vi "GetGrabberPositions.vi"(0 "reference":refnum<class "PackageNode.lvclass">, 5 "error in (no error)":errorcluster) -> (14 "reference out":refnum<class "PackageNode.lvclass">, 15 "GrabberPositions":T2[](array[typedef]) {"y" format="%.2f"; "x" format="%.2f"}, 16 "HotSpots":T1[](array[typedef]) {"HotSpot"."y" format="%.2f"; "HotSpot"."x" format="%.2f"}, 19 "error out":errorcluster)   [LabVIEW 2020, in "PackageNode.lvclass"]
doc: "public Rectangle2D getBounds(Graphics2D g2)"
uses:
  <resource>/Framework/Providers/Open_GDS/UML/PackageNode_class/PackageNode.lvclass
  C:/Program Files (x86)/National Instruments/LabVIEW 2020/resource/Framework/Providers/Open_GDS/UML/RectangularNode_class/RectangularNode.lvclass
  C:/Program Files (x86)/National Instruments/LabVIEW 2020/resource/Framework/Providers/Open_GDS/UML/AbstractNode_class/AbstractNode.lvclass
  <resource>/Framework/Providers/Open_GDS/UML/General/Point/Point Point2D.ctl
  <resource>/Framework/Providers/Open_GDS/UML/UMLEditor/UMLEditor_HotSpotData.ctl
  <resource>/Framework/Providers/Open_GDS/UML/AbstractNode_class/AbstractNode.lvclass
  <resource>/Framework/Providers/Open_GDS/UML/UMLEditor/UMLEditor_HotSpotType.ctl
  <resource>/Framework/Providers/Open_GDS/UML/RectangularNode_class/RectangularNode.lvclass
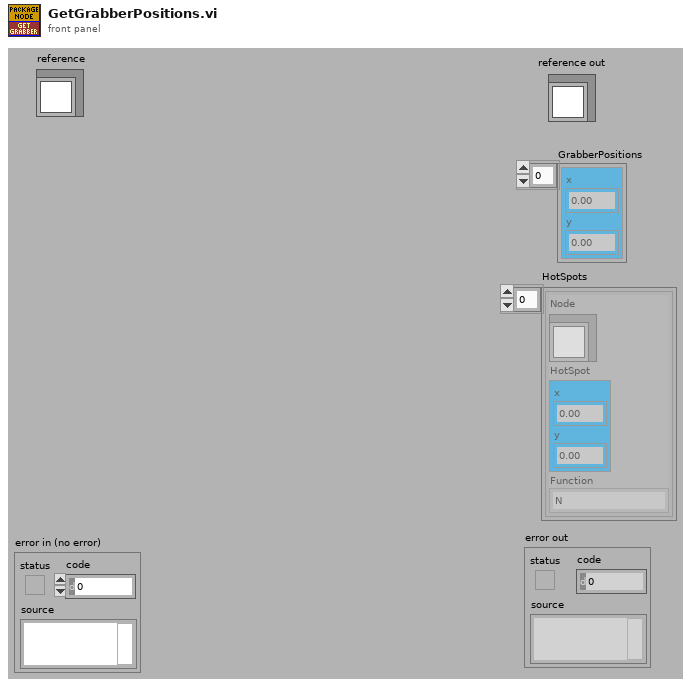
[diagram p1: front panel]
types:
  T1 = typedef "UMLEditor_HotSpotData.ctl" = cluster{"Node":refnum<class "AbstractNode.lvclass">, "HotSpot":T2, "Function":T3}
  T2 = typedef "Point Point2D.ctl" = cluster{"x":dbl, "y":dbl}
  T3 = typedef "UMLEditor_HotSpotType.ctl" = enum16{"N", "NE", "E", "SE", "S", "SW", "W", "NW", "Expand", "Collaps"}
  T4 = typedef "PackageNode.lvclass/ObjectAttributes.ctl" = cluster{"name":string, "contents":refnum<class "MultiLineString.lvclass">, "DEFAULT_TOP_WIDTH":i32, "DEFAULT_TOP_HEIGHT":i32, "DEFAULT_WIDTH":i32, "DEFAULT_HEIGHT":i32, "NAME_GAP":i32, "XGAP":i32, "YGAP":i32, "Collapsed":bool, "Note color":u32, "Justification":u16}
  T5 = typedef "RectangularNode.lvclass/ObjectAttributes.ctl" = cluster{"bounds":T6}
  T6 = typedef "Rectangle Rectangle2D.ctl" = cluster{"x":dbl, "y":dbl, "width":dbl, "height":dbl}
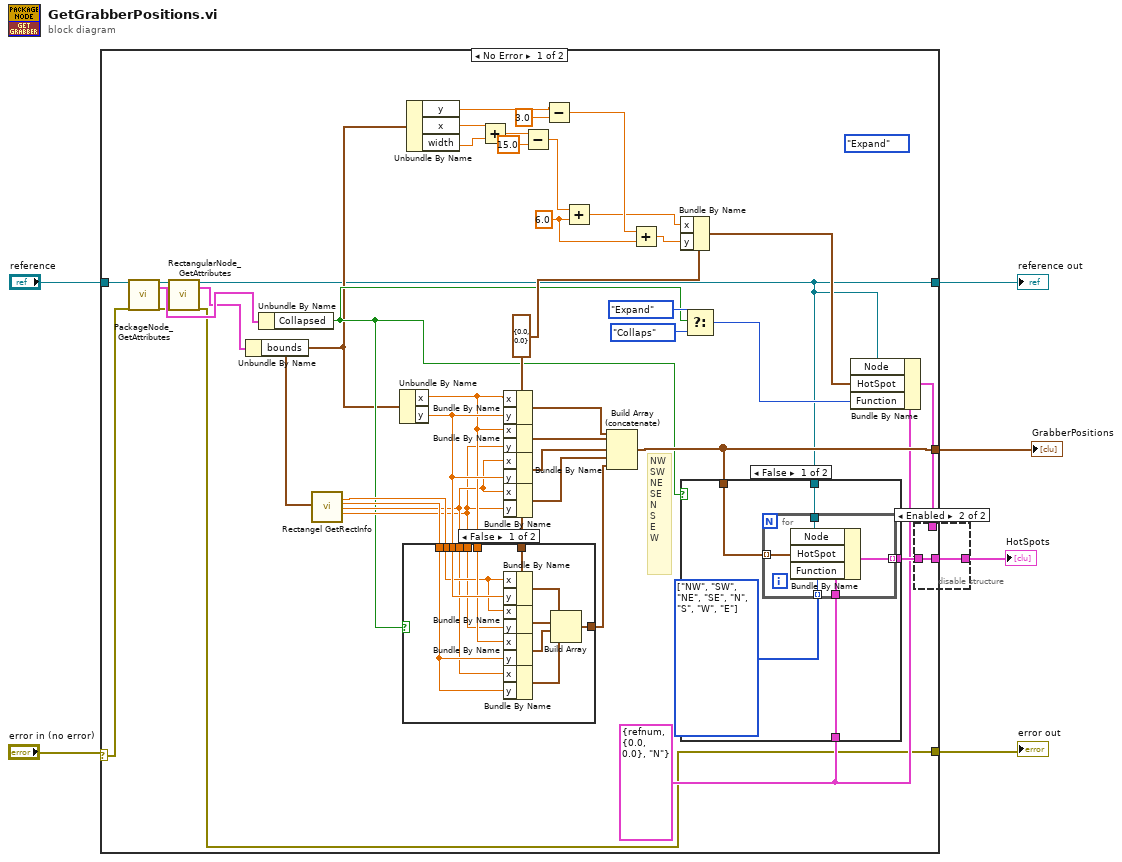
[diagram p0: block diagram]
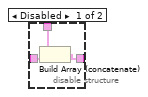
[diagram p4: hidden frame]
diagram:
  n1 = case shown="No Error" "error in (no error)" {
    selector: "error in (no error)" -> [w35 w75]
    tunnel: "reference" -> [w36 w76]
    tunnel: [w9 w75] -> w5
    tunnel: [w8 w76] -> w4
    tunnel: [w37 _] -> w2
    tunnel: [w31 _] -> w1
    frame No Error {
      w32 = T1 {"Node"=refnum, "HotSpot"={"x"=0.0, "y"=0.0}, "Function"=enum."N"} ("ObjectHotSpot")
      (unwired) UMLEditor_HotSpotType."Expand" ("Positions")
      w18 = T2 {"x"=0.0, "y"=0.0} ("point2D")
      w22 = 6.0 ("y")
      # "NW\nSW\nNE\nSE\nN\nS\nE\nW"
      n2 = call <resource>:"PackageNode_GetAttributes.vi"("reference in"=w36, "error in (no error)"=w35) -> ("reference out"=w11:refnum<class "PackageNode.lvclass">, "Data"=w12:T4, "error out"=w10:errorcluster)  [unwired: 14 in, 1 out]
      n3 = call <resource>:"RectangularNode_GetAttributes.vi"("reference in"=w11, "error in (no error)"=w10) -> ("reference out"=w8:refnum<class "PackageNode.lvclass">, "Data"=w7:T5, "error out"=w9:errorcluster)  [unwired: 14 in, 1 out]
      n4 = Unbundle By Name(w7) -> ("bounds"=w13:T6)
      n5 = Unbundle By Name(w12) -> ("Collapsed"=w14:bool)
      n6 = call <resource>:"Rectangel GetRectInfo.vi"("bounds"=w13) -> ("centerX"=w41:dbl, "centerY"=w40:dbl, "maxX"=w39:dbl, "maxY"=w38:dbl)  [unwired: 1 in, 14 out]
      n7 = Unbundle By Name(w13) -> ("x"=w42:dbl, "y"=w44:dbl)
      n8 = case shown="False" w14 {
        tunnel: w44 -> [w56 _]
        tunnel: [w55 _] -> w43
        tunnel: w42 -> [w54 _]
        tunnel: w41 -> [w53 _]
        tunnel: w40 -> [w52 _]
        tunnel: w39 -> [w51 _]
        tunnel: w38 -> [w50 _]
        tunnel: w18 -> [w49 _]
        frame False {
          n9 = Bundle By Name(cluster=w49, "x"=w53, "y"=w56) -> (w57:T2)
          n10 = Bundle By Name(cluster=w49, "x"=w53, "y"=w50) -> (w58:T2)
          n11 = Bundle By Name(cluster=w49, "x"=w54, "y"=w52) -> (w59:T2)
          n12 = Bundle By Name(cluster=w49, "x"=w51, "y"=w52) -> (w60:T2)
          n13 = Build Array(w57, w58, w59, w60) -> (w55:T2[])
        }
        frame True {
        }
      }
      n14 = Unbundle By Name(w13) -> ("y"=w21:dbl, "x"=w27:dbl, "width"=w26:dbl)
      n15 = Add(x=w27, y=w26) -> (x+y=w25:dbl)
      n16 = Bundle By Name(cluster=w18, "x"=w42, "y"=w44) -> (w48:T2)
      n17 = Bundle By Name(cluster=w18, "x"=w42, "y"=w38) -> (w47:T2)
      n18 = Bundle By Name(cluster=w18, "x"=w39, "y"=w44) -> (w46:T2)
      n19 = Bundle By Name(cluster=w18, "x"=w39, "y"=w38) -> (w45:T2)
      n20 = Subtract(x=w25, y=15.0) -> (x-y=w23:dbl)
      n21 = Subtract(x=w21, y=3.0) -> (x-y=w20:dbl)
      n22 = Add(x=w23, y=w22) -> (x+y=w17:dbl)
      n23 = Build Array (concatenate)(w48, w47, w46, w45, w43) -> (w37:T2[])
      n24 = Add(x=w20, y=w22) -> (x+y=w16:dbl)
      n25 = Bundle By Name(cluster=w18, "x"=w17, "y"=w16) -> (w15:T2)
      n26 = case shown="False" w14 {
        tunnel: w37 -> [w64 _]
        tunnel: [w63 _] -> w34
        tunnel: w32 -> [w62 _]
        tunnel: w8 -> [w61 _]
        frame False {
          w65 = T3[] [enum."NW", enum."SW", enum."NE", enum."SE", enum."N", enum."S", enum."W", enum."E"] items=["N", "NE", "E", "SE", "S", "SW", "W", "NW", "Expand", "Collaps"]
          n27 = for {
            tunnel: w62 -> [w70]
            tunnel: [w69] -> w63 mode=indexing
            tunnel: w65 -> [w68] mode=indexing
            tunnel: w64 -> [w67] mode=indexing
            tunnel: w61 -> [w66]
            n28 = Bundle By Name(cluster=w70, "Node"=w66, "HotSpot"=w67, "Function"=w68) -> (w69:T1)
          }
        }
        frame True {
        }
      }
      n29 = Select(t=UMLEditor_HotSpotType."Expand" ("Positions"), s=w14, f=UMLEditor_HotSpotType."Collaps" ("Positions")) -> (s? t:f=w28:T3)
      n30 = Bundle By Name(cluster=w32, "Node"=w8, "HotSpot"=w15, "Function"=w28) -> (w33:T1)
      n31 = disable-structure shown="Enabled" {
        disable-tunnel: w34 -> [w73 w74]
        disable-tunnel: w33 -> [w72 _]
        disable-tunnel: [w71 w74] -> w31
        frame Disabled {
          n32 = Build Array (concatenate)(w72, w73) -> (w71:T1[])
        }
        frame Enabled {
        }
      }
    }
    frame Error {
    }
  }
  "reference out" <- w4
  "error out" <- w5
  "GrabberPositions" <- w2
  "HotSpots" <- w1
